vi "Update OneOf Field Accessor.vi"(8 "error in (no error)":errorcluster, 9 "message element metadata":T1={"Field Name"="nested_message_2", "Embedded Message Name"="echo_array_NestedMessage2", "Protobuf Index"=3, "MessageElementType"=enum."MessageValue", "Repeated"=FALSE, "Is in Oneof"=TRUE, "Oneof Container Name"="echo_array_NestedMessage_union"}, 10 "class in":refnum<vi>, 11 "library in":refnum<vi>) -> (0 "error out":errorcluster)   [LabVIEW 2019, in "gRPC Template Creation Utility.lvlib"]
uses:
  gRPC Template Creation Utility.lvlib
  TypeDefs/Message Element Metadata (Scripting).ctl
  TypeDefs/Message Element Type.ctl
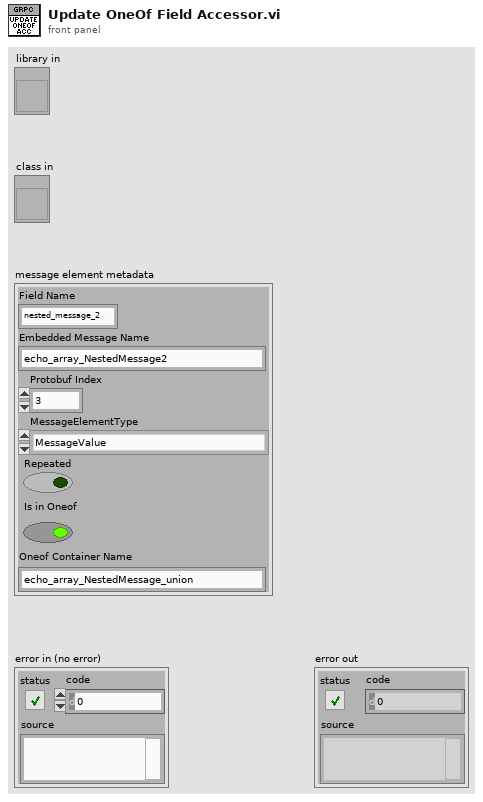
[diagram p1: front panel]
types:
  T1 = typedef "gRPC Template Creation Utility.lvlib/Message Element Metadata (Scripting).ctl" = cluster{"Field Name":string, "Embedded Message Name":string, "Protobuf Index":i32, "MessageElementType":T2, "Repeated":bool, "Is in Oneof":bool, "Oneof Container Name":string}
  T2 = typedef "gRPC Template Creation Utility.lvlib/Message Element Type.ctl" = enum32{"Int32Value", "FloatValue", "DoubleValue", "BoolValue", "StringValue", "MessageValue", "Int64Value", "UInt32Value", "UInt64Value", "EnumValue", "Bytes", "Fixed64", "Fixed32", "SFixed64", "SFixed32", "SInt64", "SInt32"}
  T3 = typedef "gRPC Template Creation Utility.lvlib/Well Known Types.ctl" = enum32{"None", "Double2DArray"}
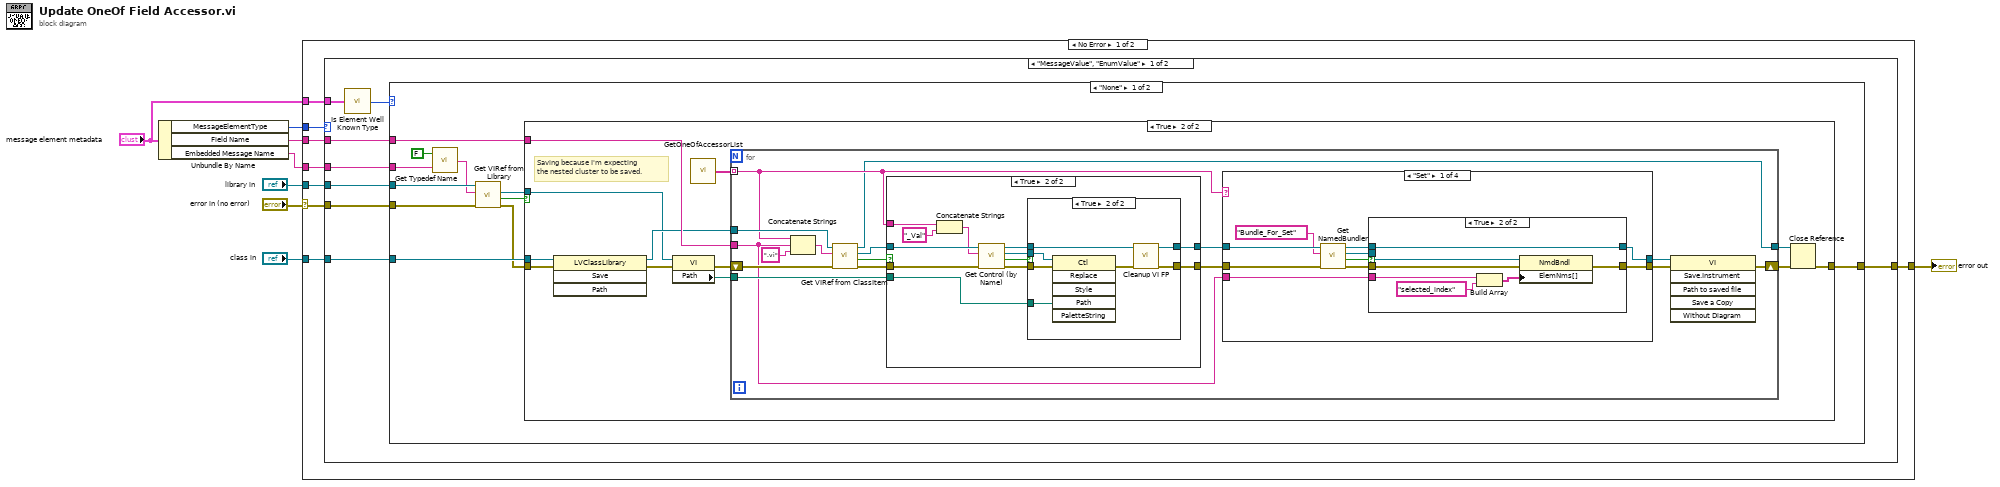
[diagram p0: block diagram]
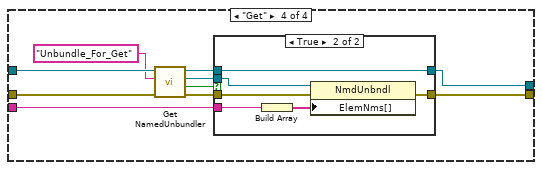
[diagram p6: hidden frame]
diagram:
  n1 = Unbundle By Name("message element metadata") -> ("MessageElementType"=w4:T2, "Field Name"=w3:string, "Embedded Message Name"=w2:string)
  n2 = case shown="No Error" "error in (no error)" {
    selector: "error in (no error)" -> [w10 w131]
    tunnel: [w16 w131] -> w8
    tunnel: w2 -> [w15 _]
    tunnel: w3 -> [w14 _]
    tunnel: "library in" -> [w13 _]
    tunnel: w4 -> [w12 _]
    tunnel: "class in" -> [w11 _]
    tunnel: "message element metadata" -> [w9 _]
    frame No Error {
      n3 = case shown="\"MessageValue\", \"EnumValue\"" w12 {
        tunnel: w10 -> [w20 w130]
        tunnel: w11 -> [w24 _]
        tunnel: w13 -> [w21 _]
        tunnel: w14 -> [w23 _]
        tunnel: w15 -> [w22 _]
        tunnel: [w19 w130] -> w16
        tunnel: w9 -> [w18 _]
        frame "MessageValue", "EnumValue" {
          n4 = call "Is Element Well Known Type.vi"("element metadata"=w18) -> ("well known type"=w17:T3)
          n5 = case shown="\"None\"" w17 {
            tunnel: w24 -> [w35 _]
            tunnel: w23 -> [w34 _]
            tunnel: w22 -> [w33 _]
            tunnel: w21 -> [w32 _]
            tunnel: w20 -> [w30 w129]
            tunnel: [w25 w129] -> w19
            frame "None" {
              n6 = call "Get Typedef Name.vi"("embedded message name"=w33, "generate serialization helpers"=FALSE ("Generate_SerializationHelper")) -> ("typedef name"=w31:string)
              n7 = call "Get VIRef from Library.vi"("error in (no error)"=w30, "item name"=w31, "library in"=w32) -> ("error out"=w29:errorcluster, "found"=w28:bool, "vi"=w27:refnum<vi>)  [unwired: 5 in, 1 out]
              n8 = case shown="True" w28 {
                tunnel: w34 -> [_ w48]
                tunnel: w35 -> [_ w46]
                tunnel: w29 -> [w36 w44]
                tunnel: [w36 w42] -> w25
                tunnel: w27 -> [_ w40]
                frame False {
                }
                frame True {
                  # "Saving because I'm expecting\nthe nested cluster to be saved."
                  n9 = invoke class="LVClassLibrary" method="Save"(reference=w46, error in=w44) -> (reference out=w45:refnum<vi>, error out=w38:errorcluster)  [unwired: 2 in, 2 out]
                  n10 = property class="VI"(reference=w40, error in=w38) -> (error out=w37:errorcluster, "Path"=w39:path)  [unwired: 1 out]
                  n11 = call "GetOneOfAccessorList.vi"() -> ("Array"=w47:string[])
                  n12 = for {
                    tunnel: w47 -> [w54] mode=indexing
                    tunnel: w48 -> [w53]
                    tunnel: w45 -> [w63]
                    tunnel: w39 -> [w59]
                    shift-right: [w49] -> w41
                    shift-left: w37 -> [w57]
                    tunnel: [w50] -> w43
                    n13 = Concatenate Strings(w54, w53, ".vi" ("string")) -> (w62:string)
                    n14 = call "Get VIRef from ClassItem.vi"("error in (no error)"=w57, "item name"=w62, "class in"=w63) -> ("error out"=w58:errorcluster, "found"=w61:bool, "vi"=w60:refnum<vi>, "class out"=w50:refnum<vi>)  [unwired: 5 in]
                    n15 = case shown="True" w61 {
                      tunnel: w60 -> [w107 w117]
                      tunnel: w54 -> [_ w118]
                      tunnel: w59 -> [_ w114]
                      tunnel: w58 -> [w106 w112]
                      tunnel: [w107 w108] -> w56
                      tunnel: [w106 w110] -> w55
                      frame False {
                      }
                      frame True {
                        n16 = Concatenate Strings(w118, "_Val" ("string")) -> (w111:string)
                        n17 = call "Get Control (by Name).vi"("error in (no error)"=w112, "Control Label"=w111, "Owner VI in"=w117) -> ("error out"=w113:errorcluster, "Found ?"=w116:bool, "Control Refnum"=w115:refnum<vi>, "Owner VI out"=w109:refnum<vi>)  [unwired: 5 in]
                        n18 = case shown="True" w116 {
                          tunnel: w115 -> [_ w128]
                          tunnel: w114 -> [_ w127]
                          tunnel: w113 -> [w121 w126]
                          tunnel: [w121 w124] -> w110
                          tunnel: w109 -> [w120 w123]
                          tunnel: [w120 w122] -> w108
                          frame False {
                            # "This will not be found for Has<Field>.vi"
                          }
                          frame True {
                            n19 = invoke class="Ctl" method="Replace"(reference=w128, error in=w126, "Path"=w127) -> (error out=w125:errorcluster)  [unwired: 3 in, 5 out]
                            n20 = call "Cleanup VI FP.vi"("error in"=w125, "vi in"=w123) -> ("error out"=w124:errorcluster, "vi out"=w122:refnum<vi>)  [unwired: 8 in]
                          }
                        }
                      }
                    }
                    n21 = case shown="\"Set\"" w54 {
                      tunnel: w56 -> [w74 w84 w86 w97]
                      tunnel: w55 -> [w72 w85 w87 w95]
                      tunnel: w53 -> [w69 _ _ w92]
                      tunnel: [w67 w85 w87 w90] -> w52
                      tunnel: [w65 w84 w86 w88] -> w51
                      frame "Set" {
                        n22 = call "Get NamedBundler.vi"("error in (no error)"=w72, "Label"="Bundle_For_Set", "Owner VI in"=w74) -> ("error out"=w68:errorcluster, "Found ?"=w71:bool, "NamedBundler ref out"=w70:refnum<vi>, "Owner VI out"=w66:refnum<vi>)  [unwired: 5 in]
                        n23 = case shown="True" w71 {
                          tunnel: w70 -> [_ w83]
                          tunnel: w69 -> [_ w81]
                          tunnel: w68 -> [w76 w79]
                          tunnel: [w76 w78] -> w67
                          tunnel: w66 -> [w75 w77]
                          tunnel: [w75 w77] -> w65
                          frame False {
                          }
                          frame True {
                            n24 = Build Array(w81, "selected_index" ("element")) -> (w82:string[])
                            n25 = property class="NmdBndl"(reference=w83, error in=w79, "ElemNms[]"=w82) -> (error out=w78:errorcluster)  [unwired: 1 out]
                          }
                        }
                      }
                      frame "Has" {
                      }
                      frame Default {
                      }
                      frame "Get" {
                        n26 = call "Get NamedUnbundler.vi"("error in (no error)"=w95, "Label"="Unbundle_For_Get", "Owner VI in"=w97) -> ("error out"=w91:errorcluster, "Found ?"=w94:bool, "NamedUnbundler ref out"=w93:refnum<vi>, "Owner VI out"=w89:refnum<vi>)  [unwired: 5 in]
                        n27 = case shown="True" w94 {
                          tunnel: w93 -> [_ w105]
                          tunnel: w92 -> [_ w103]
                          tunnel: w91 -> [w99 w102]
                          tunnel: [w99 w101] -> w90
                          tunnel: w89 -> [w98 w100]
                          tunnel: [w98 w100] -> w88
                          frame False {
                          }
                          frame True {
                            n28 = Build Array(w103) -> (w104:string[])
                            n29 = property class="NmdUnbndl"(reference=w105, error in=w102, "ElemNms[]"=w104) -> (error out=w101:errorcluster)  [unwired: 1 out]
                          }
                        }
                      }
                    }
                    n30 = invoke class="VI" method="Save.Instrument"(reference=w51, error in=w52) -> (error out=w49:errorcluster)  [unwired: 4 in, 5 out]
                  }
                  n31 = Close Reference(reference=w43, error in (no error)=w41) -> (error out=w42:errorcluster)
                }
              }
            }
            frame Default {
            }
          }
        }
        frame Default {
        }
      }
    }
    frame Error {
    }
  }
  "error out" <- w8
